vi "DAQ_Reset.vi"(8 "error in":errorcluster) -> (0 "error out":errorcluster)   [LabVIEW 2013]
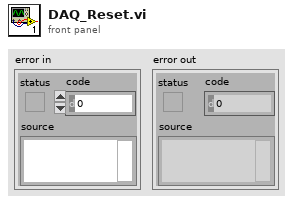
[diagram p1: front panel]
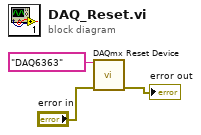
[diagram p0: block diagram]
diagram:
  n1 = call <vilib>:"DAQmx Reset Device.vi"("device in"=tag "DAQ6363", "error in"="error in") -> ("error out"=→"error out":errorcluster)  [unwired: 13 in]
